vi "Space out tunnels.vi"(8 "error in (no error)":errorcluster, 11 "Structure":refnum<vi>) -> (0 "error out":errorcluster, 1 "Tunnels out":refnum<vi>[](array[refnum]), 2 "Tunnels in":refnum<vi>[](array[refnum]), 3 "Structure out":refnum<vi>)   [LabVIEW 2012, in "Scripting Tools.lvlib"]
doc: "Spaces out the wire tunnels for the referenced G Structure. Returns arrays of references to all the tunnels in and out of the structure."
uses:
  Scripting Tools.lvlib
  <vilib>/Utility/miscctls.llb/LVPositionTypeDef.ctl
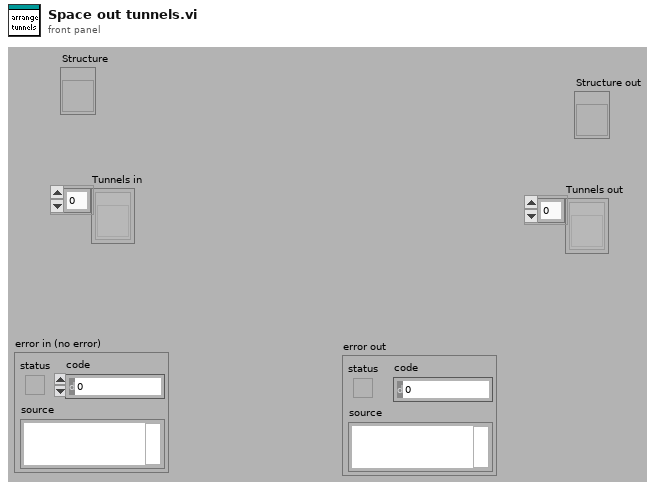
[diagram p1: front panel]
types:
  T1 = typedef "LVPositionTypeDef.ctl" = cluster{"Left":i32, "Top":i32}
  T2 = typedef "LVRectTypeDef.ctl" = cluster{"Left":i16, "Top":i16, "Right":i16, "Bottom":i16}
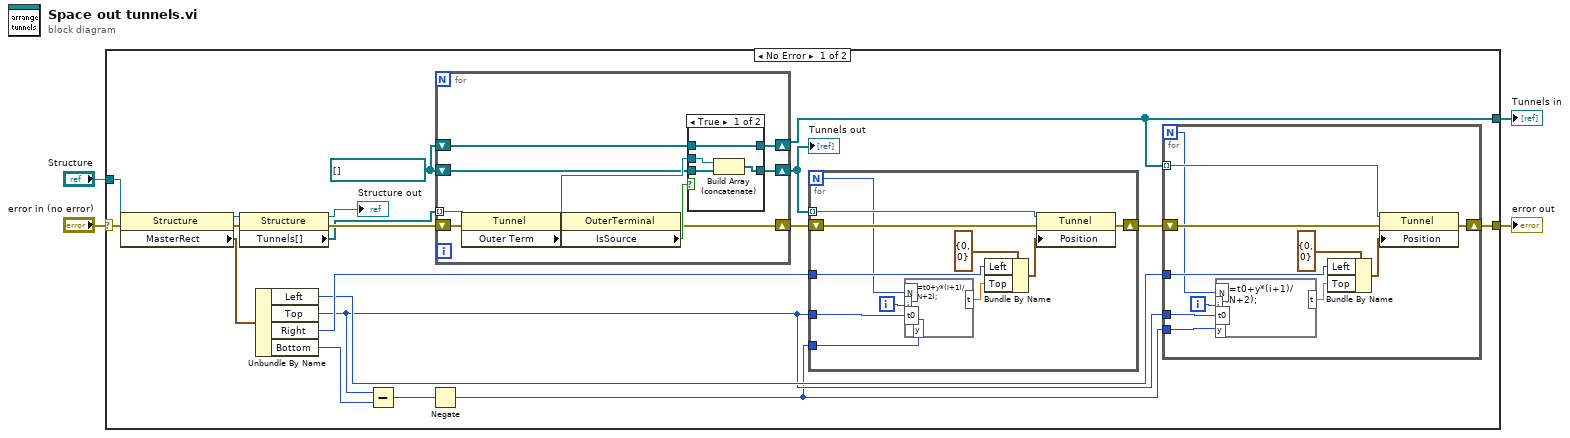
[diagram p0: block diagram]
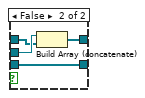
[diagram p2: hidden frame]
diagram:
  n1 = case shown="No Error" "error in (no error)" {
    selector: "error in (no error)" -> [w5 w66]
    tunnel: [w18 _] -> w4
    tunnel: [w17 w66] -> w3
    tunnel: "Structure" -> [w12 _]
    frame No Error {
      w22 = refnum<vi>[] []
      n2 = property on="Property Node" class="Structure"(reference=w12, error in=w5) -> (reference out=w15:refnum<vi>, error out=w14:errorcluster, "MasterRect"=w13:T2)
      n3 = property on="Property Node" class="Structure"(reference=w15, error in=w14) -> (reference out=→"Structure out":refnum<vi>, error out=w24:errorcluster, "Tunnels[]"=w23:refnum<vi>[])
      n4 = Unbundle By Name(w13) -> ("Left"=w8:i16, "Top"=w7:i16, "Right"=w10:i16, "Bottom"=w11:i16)
      n5 = Subtract(x=w7, y=w11) -> (x-y=w9:i16)
      n6 = Negate(x=w9) -> (-x=w6:i16)
      n7 = for {
        shift-right: [w51] -> w20
        shift-left: w22 -> [w50]
        shift-right: [w49] -> w18
        shift-left: w22 -> [w48]
        shift-right: [w47] -> w21
        shift-left: w24 -> [w56]
        tunnel: w23 -> [w57] mode=indexing
        n8 = property on="Property Node" class="Tunnel"(reference=w57, error in=w56) -> (reference out=w52:refnum<vi>, error out=w54:errorcluster, "Outer Term"=w55:refnum<vi>)
        n9 = property on="Property Node" class="OuterTerminal"(reference=w55, error in=w54) -> (error out=w47:errorcluster, "IsSource"=w53:bool)  [unwired: 1 out]
        n10 = case shown="True" w53 {
          tunnel: w52 -> [w61 w65]
          tunnel: [w60 w64] -> w51
          tunnel: w50 -> [w59 w64]
          tunnel: [w58 w63] -> w49
          tunnel: w48 -> [w58 w62]
          frame True {
            n11 = Build Array (concatenate)(w61, w59) -> (w60:refnum<vi>[])
          }
          frame False {
            n12 = Build Array (concatenate)(w65, w62) -> (w63:refnum<vi>[])
          }
        }
      }
      "Tunnels out" <- w20
      n13 = for {
        N -> [w40]
        shift-right: [w42] -> w19
        shift-left: w21 -> [w45]
        tunnel: w10 -> [w43]
        tunnel: w6 -> [w38]
        tunnel: w20 -> [w46] mode=indexing
        tunnel: w7 -> [w36]
        i -> [w39]
        n14 = formula code="t=t0+y*(i+1)/(N+2);"("N"=w40, "i"=w39, "y"=w38, "t0"=w36) -> ("t"=w37:dbl)
        n15 = Bundle By Name(cluster=T1 {"Left"=0, "Top"=0} ("Position"), "Left"=w43, "Top"=w37) -> (w41:T1)
        n16 = property on="Property Node" class="Tunnel"(reference=w46, error in=w45, "Position"=w41) -> (error out=w42:errorcluster)  [unwired: 1 out]
      }
      n17 = for {
        N -> [w29]
        shift-right: [w32] -> w17
        shift-left: w19 -> [w34]
        tunnel: w8 -> [w30]
        tunnel: w6 -> [w27]
        tunnel: w18 -> [w35] mode=indexing
        tunnel: w7 -> [w26]
        i -> [w28]
        n18 = formula code="t=t0+y*(i+1)/(N+2);"("N"=w29, "i"=w28, "y"=w27, "t0"=w26) -> ("t"=w25:dbl)
        n19 = Bundle By Name(cluster=T1 {"Left"=0, "Top"=0} ("Position"), "Left"=w30, "Top"=w25) -> (w31:T1)
        n20 = property on="Property Node" class="Tunnel"(reference=w35, error in=w34, "Position"=w31) -> (error out=w32:errorcluster)  [unwired: 1 out]
      }
    }
    frame Error {
    }
  }
  "error out" <- w3
  "Tunnels in" <- w4
